vi "GOOP_GetOverrideMethods.vi"(1 "LvClassItem":refnum<vi>, 5 "error in (no error)":errorcluster) -> (12 "IsMustOverrideVI":bool[](array[boolean]), 13 "IsAPropertyDefinitionVI":bool[](array[boolean]), 15 "DynamicMethods(Names)":string[](array[string]), 16 "DynamicMehods(Paths)":path[](array[path]), 17 "Scope":T1(array[ring]), 18 "ConnectorPaneHeight":i32[](array[numeric]), 19 "error out":errorcluster)   [LabVIEW 2020]
panel:
  # "0 or -1 means Full Icon height\n1 is only one connector terminal height\n  and the header is then removed."
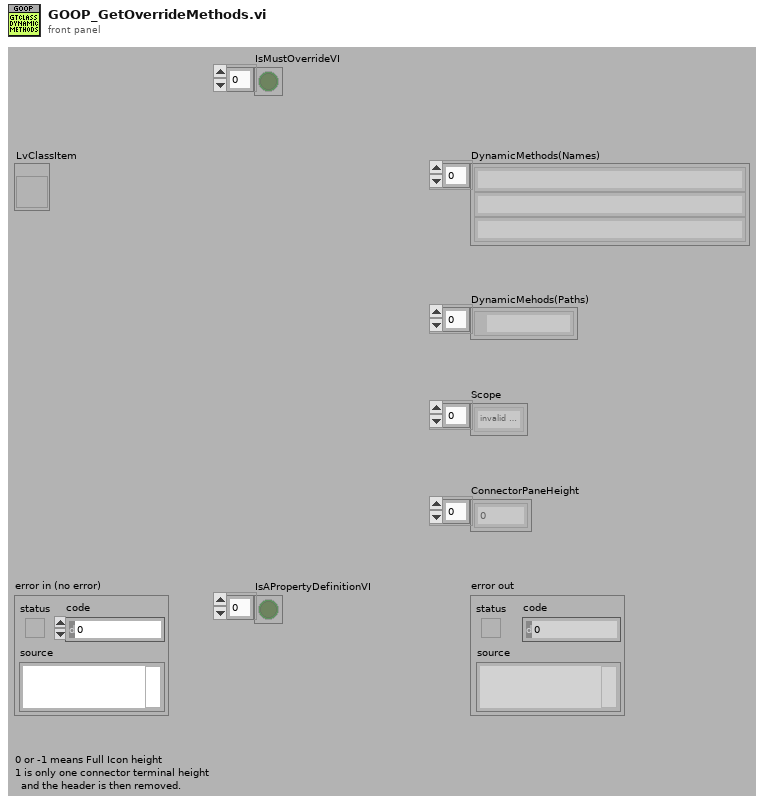
[diagram p1: front panel]
types:
  T1 = enum32{"invalid scope", "public", "private", "protected", "community"}[]
  T2 = cluster{string, "Path":path, "Source Scope:Get":enum32{"invalid scope", "public", "private", "protected", "community"}, "Numeric":i32, bool, bool}[]
  T3 = enum32{"invalid scope", "public", "private", "protected", "community"}
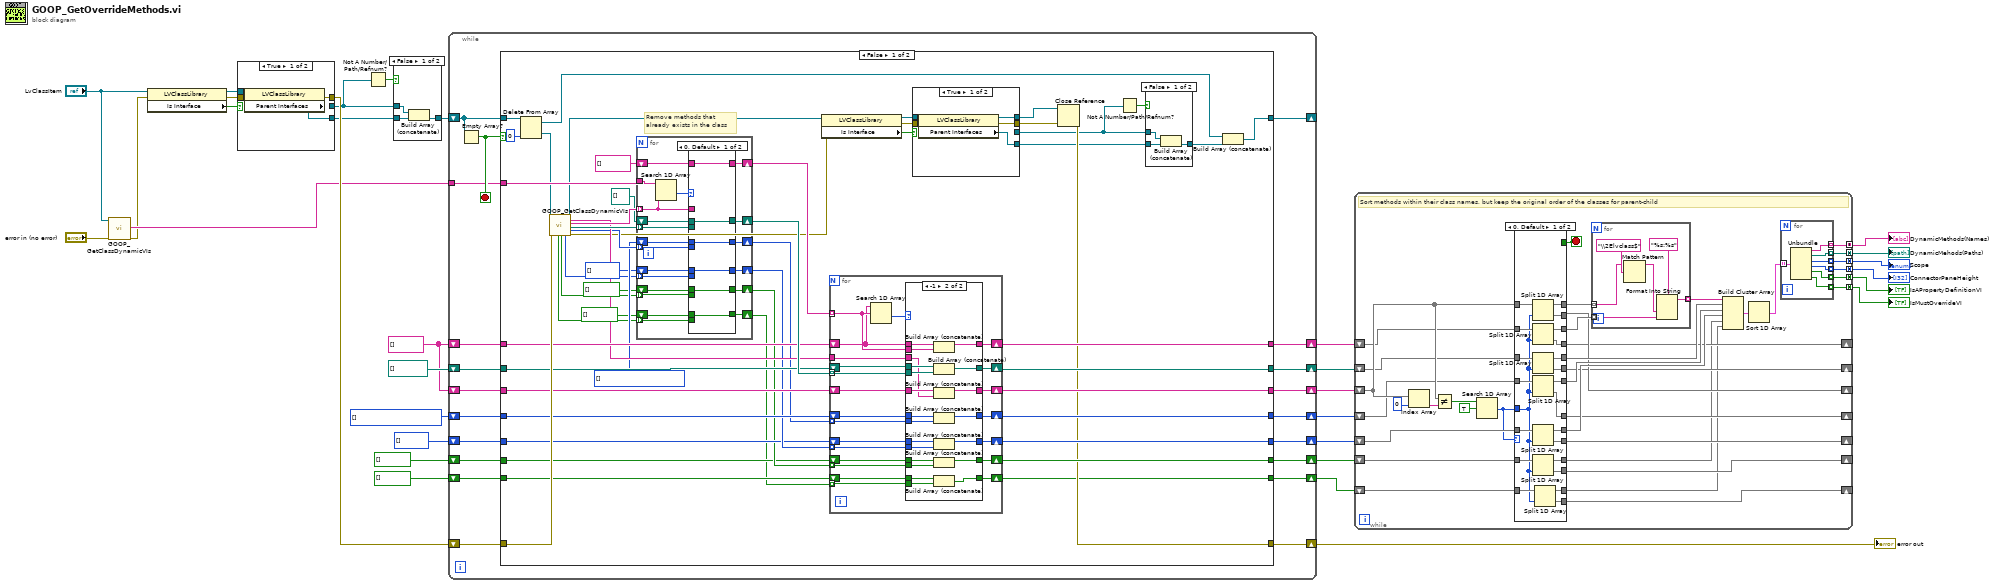
[diagram p0: block diagram]
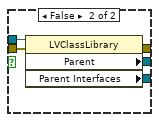
[diagram p2: hidden frame]
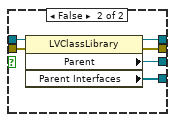
[diagram p4: hidden frame]
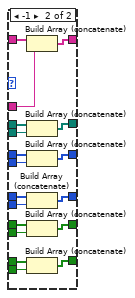
[diagram p5: hidden frame]
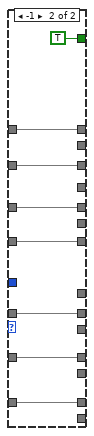
[diagram p9: hidden frame]
diagram:
  w26 = T1 [] items=["invalid scope", "public", "private", "protected", "community"]
  w27 = string[] []
  n1 = call "GOOP_GetClassDynamicVIs.vi"("LvClassIn"="LvClassItem", "error in"="error in (no error)") -> ("VINames(without Prefix)"=w29:string[], "error out"=w6:errorcluster)  [unwired: 9 in, 7 out]
  n2 = property class="LVClassLibrary"(reference="LvClassItem", error in=w6) -> (reference out=w7:refnum<vi>, error out=w5:errorcluster, "Is Interface"=w4:bool)
  n3 = case shown="True" w4 {
    tunnel: [w36 w41] -> w32
    tunnel: [w35 w40] -> w12
    tunnel: [_ w39] -> w10
    tunnel: w7 -> [w34 w38]
    tunnel: w5 -> [w33 w37]
    frame True {
      n4 = property class="LVClassLibrary"(reference=w34, error in=w33) -> (error out=w36:errorcluster, "Parent Interfaces"=w35:refnum<vi>[])  [unwired: 1 out]
    }
    frame False {
      n5 = property class="LVClassLibrary"(reference=w38, error in=w37) -> (error out=w41:errorcluster, "Parent"=w39:refnum<vi>, "Parent Interfaces"=w40:refnum<vi>[])  [unwired: 1 out]
    }
  }
  n6 = Not A Number/Path/Refnum?(number/path/refnum=w10) -> (NaN/Path/Refnum?=w9:bool)
  n7 = case shown="False" w9 {
    tunnel: w12 -> [w44 w45]
    tunnel: [w43 w45] -> w11
    tunnel: w10 -> [w42 _]
    frame False {
      n8 = Build Array (concatenate)(w42, w44) -> (w43:refnum<vi>[])
    }
    frame True {
    }
  }
  n9 = while {
    shift-right: [w63] -> _
    shift-left: w11 -> [w64]
    shift-right: [w62] -> w31
    shift-left: w32 -> [w61]
    shift-right: [w59] -> w23
    shift-left: w27 -> [w60]
    tunnel: w29 -> [w58]
    shift-right: [w56] -> w21
    shift-left: path[] [] -> [w57]
    shift-right: [w54] -> w24
    shift-left: w27 -> [w55]
    shift-right: [w52] -> w19
    shift-left: w26 -> [w53]
    shift-right: [w51] -> w17
    shift-left: i32[] [] -> [w50]
    shift-right: [w48] -> w14
    shift-left: bool[] [] -> [w49]
    shift-right: [w46] -> w2
    shift-left: bool[] [] -> [w47]
    stop <- w65 stop-if-true
    n10 = Empty Array?(array=w64) -> (empty?=w65:bool)
    n11 = case shown="False" w65 {
      tunnel: w64 -> [w85 w235]
      tunnel: [w80 w235] -> w63
      tunnel: [w81 w234] -> w62
      tunnel: w61 -> [w117 w234]
      tunnel: w60 -> [w110 w233]
      tunnel: [w109 w233] -> w59
      tunnel: w58 -> [w116 _]
      tunnel: w57 -> [w108 w232]
      tunnel: [w107 w232] -> w56
      tunnel: w55 -> [w105 w231]
      tunnel: [w104 w231] -> w54
      tunnel: w53 -> [w100 w230]
      tunnel: [w98 w230] -> w52
      tunnel: [w94 w229] -> w51
      tunnel: w50 -> [w93 w229]
      tunnel: w49 -> [w89 w228]
      tunnel: [w88 w228] -> w48
      tunnel: w47 -> [w68 w227]
      tunnel: [w66 w227] -> w46
      frame False {
        w101 = T1 [] items=["invalid scope", "public", "private", "protected", "community"]
        # "Remove methods that\nalready exists in the class"
        n12 = Delete From Array(array=w85, index=0) -> (deleted portion=w86:refnum<vi>, array with subset deleted=w82:refnum<vi>[])  [unwired: 1 in]
        n13 = call "GOOP_GetClassDynamicVIs.vi"("LvClassIn"=w86, "error in"=w117) -> ("IsMustOverride"=w70:bool[], "IsAPropertyDefinitionVI"=w92:bool[], "ConnectorPaneHeight"=w97:i32[], "LvClassOut"=w76:refnum<vi>, "ClassName"=w106:string, "VINames(without Prefix)"=w115:string[], "ViPaths"=w112:path[], "Scope"=w102:T1, "error out"=w75:errorcluster)  [unwired: 9 in]
        n14 = for {
          tunnel: w116 -> [w148]
          tunnel: w115 -> [w144] mode=indexing
          shift-right: [w145] -> w113
          shift-left: string[] [] -> [w146]
          shift-right: [w141] -> w111
          shift-left: path[] [] -> [w143]
          tunnel: w112 -> [w142] mode=indexing
          shift-right: [w138] -> w99
          shift-left: w101 -> [w140]
          tunnel: w102 -> [w139] mode=indexing
          shift-right: [w137] -> w95
          shift-left: i32[] [] -> [w135]
          tunnel: w97 -> [w136] mode=indexing
          shift-right: [w132] -> w90
          shift-left: bool[] [] -> [w134]
          tunnel: w92 -> [w133] mode=indexing
          tunnel: w70 -> [w130] mode=indexing
          shift-right: [w131] -> w67
          shift-left: bool[] [] -> [w129]
          n15 = Search 1D Array(1D array=w148, element=w144) -> (index of element=w147:i32)  [unwired: 1 in]
          n16 = case shown="0, Default" w147 {
            tunnel: w146 -> [w154 w172]
            tunnel: [w154 w171] -> w145
            tunnel: w144 -> [_ w170]
            tunnel: w143 -> [w153 w169]
            tunnel: w142 -> [_ w168]
            tunnel: [w153 w167] -> w141
            tunnel: w140 -> [w152 w166]
            tunnel: w139 -> [_ w165]
            tunnel: [w152 w164] -> w138
            tunnel: w135 -> [w151 w161]
            tunnel: w136 -> [_ w162]
            tunnel: [w151 w163] -> w137
            tunnel: w134 -> [w150 w160]
            tunnel: w133 -> [_ w159]
            tunnel: [w150 w158] -> w132
            tunnel: [w149 w156] -> w131
            tunnel: w130 -> [_ w157]
            tunnel: w129 -> [w149 w155]
            frame 0, Default {
            }
            frame -1 {
              n17 = Build Array (concatenate)(w172, w170) -> (w171:string[])
              n18 = Build Array (concatenate)(w169, w168) -> (w167:path[])
              n19 = Build Array (concatenate)(w166, w165) -> (w164:T1)
              n20 = Build Array (concatenate)(w161, w162) -> (w163:i32[])
              n21 = Build Array (concatenate)(w160, w159) -> (w158:bool[])
              n22 = Build Array (concatenate)(w155, w157) -> (w156:bool[])
            }
          }
        }
        n23 = property class="LVClassLibrary"(reference=w76, error in=w75) -> (reference out=w77:refnum<vi>, error out=w78:errorcluster, "Is Interface"=w79:bool)
        n24 = for {
          tunnel: w113 -> [w193] mode=indexing
          tunnel: w111 -> [w192] mode=indexing
          shift-right: [w190] -> w109
          shift-left: w110 -> [w191]
          shift-right: [w188] -> w107
          shift-left: w108 -> [w189]
          tunnel: w106 -> [w187]
          shift-right: [w185] -> w104
          shift-left: w105 -> [w186]
          shift-right: [w182] -> w98
          shift-left: w100 -> [w184]
          tunnel: w99 -> [w183] mode=indexing
          shift-right: [w181] -> w94
          shift-left: w93 -> [w179]
          tunnel: w95 -> [w180] mode=indexing
          shift-right: [w176] -> w88
          shift-left: w89 -> [w178]
          tunnel: w90 -> [w177] mode=indexing
          shift-right: [w174] -> w66
          shift-left: w68 -> [w175]
          tunnel: w67 -> [w173] mode=indexing
          n25 = Search 1D Array(1D array=w191, element=w193) -> (index of element=w194:i32)  [unwired: 1 in]
          n26 = case shown="-1" w194 {
            tunnel: w191 -> [w201 w222]
            tunnel: [w201 w221] -> w190
            tunnel: w193 -> [_ w215]
            tunnel: w192 -> [_ w220]
            tunnel: w189 -> [w200 w219]
            tunnel: [w200 w218] -> w188
            tunnel: w187 -> [_ w216]
            tunnel: w186 -> [w199 w217]
            tunnel: [w199 w214] -> w185
            tunnel: w184 -> [w198 w213]
            tunnel: w183 -> [_ w212]
            tunnel: [w198 w211] -> w182
            tunnel: w179 -> [w197 w208]
            tunnel: w180 -> [_ w209]
            tunnel: [w197 w210] -> w181
            tunnel: w178 -> [w196 w207]
            tunnel: w177 -> [_ w206]
            tunnel: [w196 w205] -> w176
            tunnel: w173 -> [_ w204]
            tunnel: [w195 w203] -> w174
            tunnel: w175 -> [w195 w202]
            frame 0, Default {
            }
            frame -1 {
              n27 = Build Array (concatenate)(w222, w215) -> (w221:string[])
              n28 = Build Array (concatenate)(w219, w220) -> (w218:path[])
              n29 = Build Array (concatenate)(w217, w216) -> (w214:string[])
              n30 = Build Array (concatenate)(w213, w212) -> (w211:T1)
              n31 = Build Array (concatenate)(w208, w209) -> (w210:i32[])
              n32 = Build Array (concatenate)(w207, w206) -> (w205:bool[])
              n33 = Build Array (concatenate)(w202, w204) -> (w203:bool[])
            }
          }
        }
        n34 = case shown="True" w79 {
          tunnel: [w122 w128] -> w74
          tunnel: [w121 w127] -> w71
          tunnel: [_ w126] -> w72
          tunnel: w77 -> [w120 w125]
          tunnel: w78 -> [w119 w124]
          tunnel: [w118 w123] -> w73
          frame True {
            n35 = property class="LVClassLibrary"(reference=w120, error in=w119) -> (reference out=w118:refnum<vi>, error out=w122:errorcluster, "Parent Interfaces"=w121:refnum<vi>[])
          }
          frame False {
            n36 = property class="LVClassLibrary"(reference=w125, error in=w124) -> (reference out=w123:refnum<vi>, error out=w128:errorcluster, "Parent"=w126:refnum<vi>, "Parent Interfaces"=w127:refnum<vi>[])
          }
        }
        n37 = Close Reference(reference=w73, error in (no error)=w74) -> (error out=w81:errorcluster)
        n38 = Not A Number/Path/Refnum?(number/path/refnum=w72) -> (NaN/Path/Refnum?=w84:bool)
        n39 = case shown="False" w84 {
          tunnel: w71 -> [w225 w226]
          tunnel: [w224 w226] -> w83
          tunnel: w72 -> [w223 _]
          frame False {
            n40 = Build Array (concatenate)(w223, w225) -> (w224:refnum<vi>[])
          }
          frame True {
          }
        }
        n41 = Build Array (concatenate)(w82, w83) -> (w80:refnum<vi>[])
      }
      frame True {
      }
    }
  }
  "error out" <- w31
  n42 = while {
    tunnel: [w257] -> w22 mode=concatenating
    tunnel: [w255] -> w20 mode=concatenating
    tunnel: [w253] -> w18 mode=concatenating
    tunnel: [w251] -> w16 mode=concatenating
    shift-right: [w250] -> _
    shift-left: w24 -> [w267]
    shift-right: [w249] -> _
    shift-left: w23 -> [w265]
    shift-right: [w248] -> _
    shift-left: w21 -> [w256]
    shift-right: [w247] -> _
    shift-left: w19 -> [w254]
    shift-right: [w246] -> _
    shift-left: w17 -> [w252]
    shift-right: [w243] -> _
    shift-left: w14 -> [w242]
    tunnel: [w240] -> w13 mode=concatenating
    shift-right: [w237] -> _
    shift-left: w2 -> [w238]
    tunnel: [w236] -> w1 mode=concatenating
    stop <- w244 stop-if-true
    # "Sort methods within their class names, but keep the original order of the classes for parent-child"
    n43 = Index Array(array=w267, index=0) -> (element=w270:string)
    n44 = Not Equal?(x=w267, y=w270) -> (x != y?=w269:bool[])
    n45 = Search 1D Array(1D array=w269, element=TRUE) -> (index of element=w245:i32)  [unwired: 1 in]
    n46 = case shown="0, Default" w245 {
      tunnel: w245 -> [w272 _]
      tunnel: w267 -> [w293 w301]
      tunnel: [w292 w301] -> w266
      tunnel: w265 -> [w291 w300]
      tunnel: [w290 w300] -> w264
      tunnel: [w289 w299] -> w263
      tunnel: [w288 w298] -> w262
      tunnel: [w287 w297] -> w261
      tunnel: w256 -> [w286 w299]
      tunnel: w254 -> [w285 w298]
      tunnel: w252 -> [w284 w297]
      tunnel: [w283 _] -> w250
      tunnel: [w282 _] -> w249
      tunnel: [w281 _] -> w248
      tunnel: [w280 _] -> w247
      tunnel: [w279 _] -> w246
      tunnel: [_ TRUE] -> w244
      tunnel: [w278 w295] -> w241
      tunnel: [w276 _] -> w243
      tunnel: w242 -> [w277 w295]
      tunnel: [w275 w294] -> w239
      tunnel: w238 -> [w274 w294]
      tunnel: [w273 _] -> w237
      frame 0, Default {
        n47 = Split 1D Array(array=w293, index=w272) -> (first subarray=w292:string[], second subarray=w283:string[])
        n48 = Split 1D Array(array=w291, index=w272) -> (first subarray=w290:string[], second subarray=w282:string[])
        n49 = Split 1D Array(array=w286, index=w272) -> (first subarray=w289:path[], second subarray=w281:path[])
        n50 = Split 1D Array(array=w285, index=w272) -> (first subarray=w288:T1, second subarray=w280:T1)
        n51 = Split 1D Array(array=w284, index=w272) -> (first subarray=w287:i32[], second subarray=w279:i32[])
        n52 = Split 1D Array(array=w277, index=w272) -> (first subarray=w278:bool[], second subarray=w276:bool[])
        n53 = Split 1D Array(array=w274, index=w272) -> (first subarray=w275:bool[], second subarray=w273:bool[])
      }
      frame -1 {
      }
    }
    n54 = for {
      tunnel: w266 -> [w310] mode=indexing
      tunnel: w264 -> [w313] mode=indexing
      tunnel: [w312] -> w258 mode=indexing
      n55 = Match Pattern(string=w310, regular expression="\\2Elvclass$") -> (before substring=w309:string)  [unwired: 1 in, 3 out]
      n56 = Format Into String(format string="%s:%s", w309, w313) -> (resulting string=w312:string)  [unwired: 2 in, 1 out]
    }
    n57 = Build Cluster Array(w258, w263, w262, w261, w241, w239) -> (w260:T2)
    n58 = Sort 1D Array(array=w260) -> (sorted array=w259:T2)
    n59 = for {
      tunnel: w259 -> [w308] mode=indexing
      tunnel: [w307] -> w257 mode=indexing
      tunnel: [w306] -> w255 mode=indexing
      tunnel: [w305] -> w253 mode=indexing
      tunnel: [w304] -> w251 mode=indexing
      tunnel: [w303] -> w240 mode=indexing
      tunnel: [w302] -> w236 mode=indexing
      n60 = Unbundle(w308) -> (w307:string, "Path"=w306:path, "Source Scope:Get"=w305:T3, "Numeric"=w304:i32, w303:bool, w302:bool)
    }
  }
  "DynamicMethods(Names)" <- w22
  "DynamicMehods(Paths)" <- w20
  "Scope" <- w18
  "ConnectorPaneHeight" <- w16
  "IsAPropertyDefinitionVI" <- w13
  "IsMustOverrideVI" <- w1
